vi "RDV-changeRefLines.vi"(7 "Add lines for ref":bool, 8 "error in (no error)":errorcluster, 11 "RDV-Reflection_Data_viewer in":refnum<class "RDV-Reflection_Data_viewer.lvclass">) -> (0 "error out":errorcluster, 3 "RDV-Reflection_Data_viewer out":refnum<class "RDV-Reflection_Data_viewer.lvclass">)   [LabVIEW 2020, in "RDV-Reflection_Data_viewer.lvclass"]
doc: "Shows or hides the reference lines on the viewer's graphs."
uses:
  RDV-Reflection_Data_viewer.lvclass
  RDV-Reflection_Data_viewer.lvclass/RDV-Reflection_Data_viewer.ctl
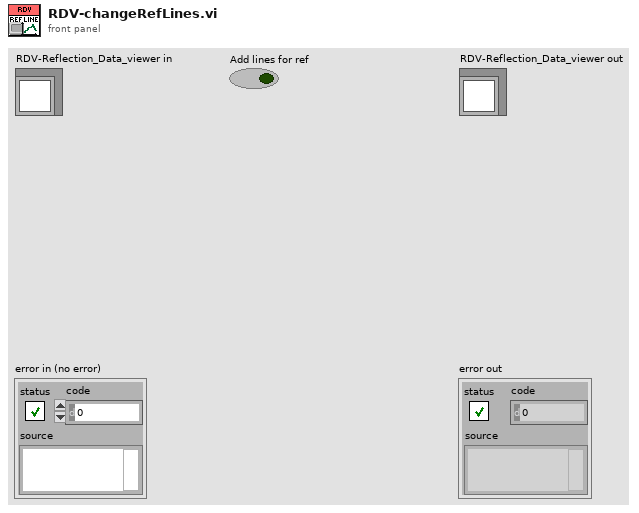
[diagram p1: front panel]
types:
  T1 = typedef "RDV-Reflection_Data_viewer.lvclass/RDV-UPDATE_IGNORE_LIST.ctl" = string[]
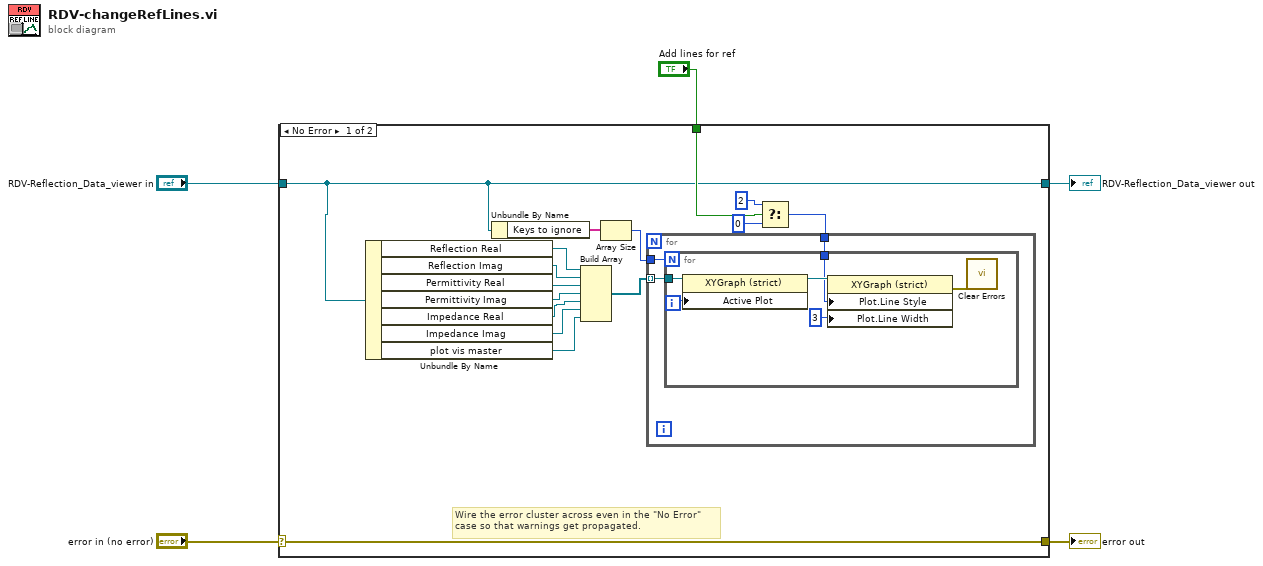
[diagram p0: block diagram]
diagram:
  n1 = case shown="No Error" "error in (no error)" {
    selector: "error in (no error)" -> [w21 w32]
    tunnel: [w21 w32] -> w4
    tunnel: [w8 w31] -> w2
    tunnel: "RDV-Reflection_Data_viewer in" -> [w8 w31]
    tunnel: "Add lines for ref" -> [w12 _]
    frame No Error {
      # "Wire the error cluster across even in the \"No Error\"\ncase so that warnings get propagated."
      n2 = Unbundle By Name(w8) -> ("Reflection Real"=w20:refnum<vi>, "Reflection Imag"=w19:refnum<vi>, "Permittivity Real"=w18:refnum<vi>, "Permittivity Imag"=w17:refnum<vi>, "Impedance Real"=w15:refnum<vi>, "Impedance Imag"=w14:refnum<vi>, "plot vis master"=w7:refnum<vi>)
      n3 = Unbundle By Name(w8) -> ("Keys to ignore"=w9:T1)
      n4 = Build Array(w20, w19, w18, w17, w15, w14, w7) -> (w16:refnum<vi>[])
      n5 = Array Size(array=w9) -> (size(s)=w6:i32)
      n6 = Select(t=u8 2 ("Cursor.Line Style"), s=w12, f=u8 0) -> (s? t:f=w10:u8)
      n7 = for {
        tunnel: w16 -> [w24] mode=indexing
        tunnel: w10 -> [w23]
        tunnel: w6 -> [w22]
        n8 = for {
          N: w22 -> [_]
          tunnel: w24 -> [w30]
          tunnel: w23 -> [w26]
          i -> [w29]
          n9 = property on="Property Node" class="XYGraph (strict)"(reference=w30, "Active Plot"=w29) -> (reference out=w28:refnum<vi>)  [unwired: 1 in, 1 out]
          n10 = property on="Property Node" class="XYGraph (strict)"(reference=w28, "Plot.Line Style"=w26, "Plot.Line Width"=u8 3) -> (error out=w27:errorcluster)  [unwired: 1 in, 1 out]
          n11 = call <vilib>:"Clear Errors.vi"("error in (no error)"=w27) -> ()  [unwired: 5 in, 2 out]
        }
      }
    }
    frame Error {
    }
  }
  "error out" <- w4
  "RDV-Reflection_Data_viewer out" <- w2
